vi "Delete Files and Directories.vi"(3 "error in":errorcluster, 4 "Items to Delete":string[](array[string]), 5 "Base path":path) -> (0 "error out":errorcluster)   [LabVIEW 2023]
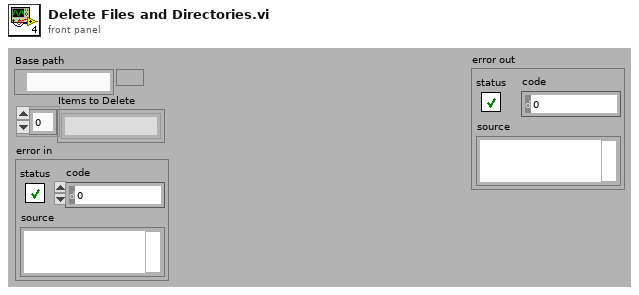
[diagram p1: front panel]
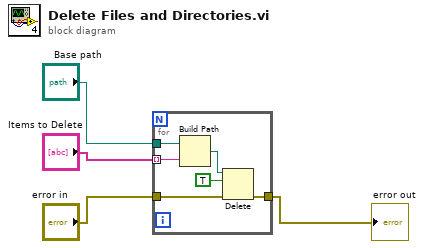
[diagram p0: block diagram]
diagram:
  n1 = for {
    tunnel: "Items to Delete" -> [w6] mode=indexing
    tunnel: "error in" -> [w8]
    tunnel: [w7] -> w4
    tunnel: "Base path" -> [w5]
    n2 = Build Path(base path=w5, name or relative path=w6) -> (appended path=w10:path)
    n3 = Delete(path (use dialog)=w10, entire hierarchy (F)=TRUE, error in=w8) -> (error out=w7:errorcluster)  [unwired: 2 in, 2 out]
  }
  "error out" <- w4
